vi "Set Result.vi"(8 "error in (no error)":errorcluster, 10 "XY Plot":refnum<vi>, 11 "3way Lap in":refnum<class "3way Lap.lvclass">) -> (0 "error out":errorcluster, 3 "3way Lap out":refnum<class "3way Lap.lvclass">)   [LabVIEW 2025, in "Flow Grind.lvlib" / "3way Lap.lvclass"]
uses:
  3way Lap.lvclass
  FG configuration/FlowGrind configuration.lvclass
  3way Lap.lvclass/3way Lap.ctl
  FG configuration/FlowGrind configuration.lvclass/FlowGrind configuration.ctl
  FG configuration/Read FlowGrind.vi
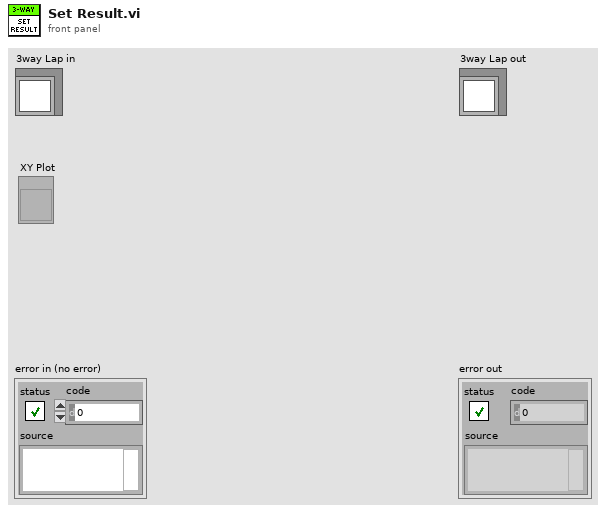
[diagram p1: front panel]
types:
  T1 = cluster{"Name":string, "Color":u32, "Style":u8, "Point Style":u8, "Name Visible":bool, "Allow Drag":bool, "Annotation Mode":u32, "Plot":i32, "Index":i32, "Position":cluster{"X":dbl, "Y":dbl}, "X Scale":u32, "Y Scale":u32, "Show Arrow":bool, "Lock Name":bool, "Plot Area":i32, "Label Offset":cluster{"X":dbl, "Y":dbl}}
  T2 = typedef "Flow Grind.lvlib/FlowGrind configuration.lvclass/FlowGrind Settings.ctl" = cluster{"Build Profile":cluster{"Ramp Start":dbl, "Ramp End":dbl, "Ramp Rate Far":dbl, "Ramp Rate Close":dbl, "Null Lower Limit":dbl, "Null Upper Limit":dbl, "Test Mode":string}[][], "Scale Factor":cluster{"X":dbl, "Y":dbl}, "Lap Condition":dbl, "Supply Pressure":dbl, "Simulated?":bool}
  T3 = typedef "LVAnnotationListTypeDef.ctl" = cluster{"Name":string, "Color":u32, "Style":u8, "Point Style":u8, "Name Visible":bool, "Allow Drag":bool, "Annotation Mode":u32, "Plot":i32, "Index":i32, "Position":cluster{"X":dbl, "Y":dbl}, "X Scale":u32, "Y Scale":u32, "Show Arrow":bool, "Lock Name":bool, "Plot Area":i32, "Label Offset":cluster{"X":dbl, "Y":dbl}}[]
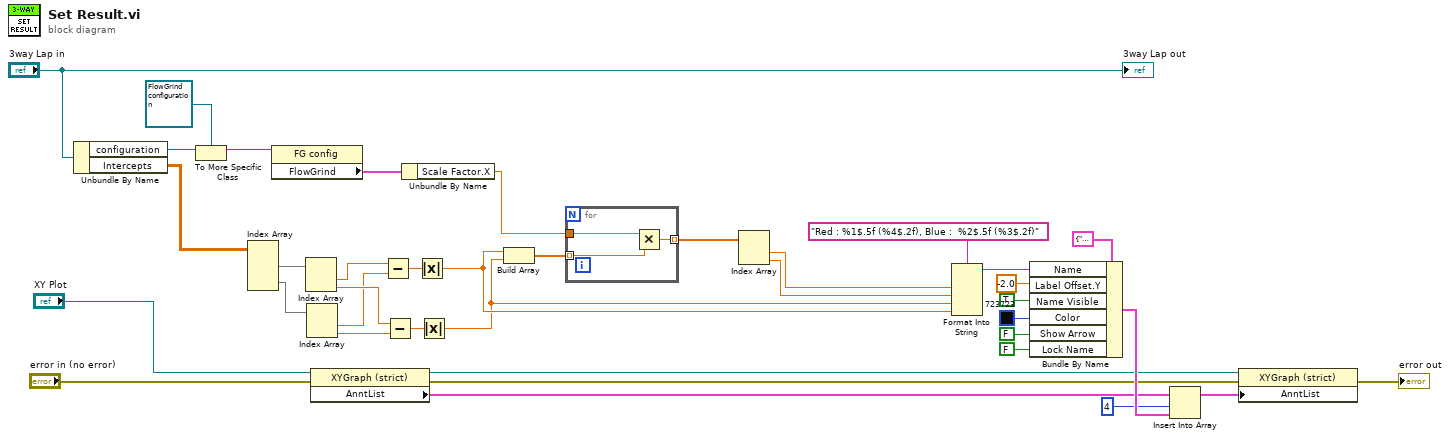
[diagram p0: block diagram]
diagram:
  n1 = Unbundle By Name("3way Lap in") -> ("configuration"=w6:refnum<class "FlowGrind configuration.lvclass">, "Intercepts"=w7:dbl[][])
  n2 = To More Specific Class(target class=refnum<class "FlowGrind configuration.lvclass"> refnum ("Flow Grind.lvlib:XY Plotter config"), reference=w6) -> (specific class reference=w4:refnum<class "FlowGrind configuration.lvclass">)  [unwired: 1 in, 1 out]
  n3 = Index Array(array=w7) -> (element #1=w13:dbl[], element #2=w14:dbl[])  [unwired: 4 in]
  n4 = property class="FG config"(reference=w4) -> ("FlowGrind"=w3:T2)  [unwired: 1 in, 2 out]
  n5 = Index Array(array=w13) -> (element #1=w15:dbl, element #2=w17:dbl)  [unwired: 2 in]
  n6 = Index Array(array=w14) -> (element #1=w16:dbl, element #2=w18:dbl)  [unwired: 2 in]
  n7 = property class="XYGraph (strict)"(reference="XY Plot", error in="error in (no error)") -> (reference out=w32:refnum<vi>, error out=w34:errorcluster, "AnntList"=w33:T3)
  n8 = Subtract(x=w15, y=w16) -> (x-y=w19:dbl)
  n9 = Subtract(x=w17, y=w18) -> (x-y=w20:dbl)
  n10 = Unbundle By Name(w3) -> ("Scale Factor.X"=w2:dbl)
  n11 = Absolute Value(x=w19) -> (abs(x)=w30:dbl)
  n12 = Absolute Value(x=w20) -> (abs(x)=w29:dbl)
  n13 = Build Array(w30, w29) -> (w11:dbl[])
  n14 = for {
    tunnel: w11 -> [w39] mode=indexing
    tunnel: w2 -> [w41]
    tunnel: [w40] -> w31 mode=indexing
    n15 = Multiply(x=w41, y=w39) -> (x*y=w40:dbl)
  }
  n16 = Index Array(array=w31) -> (element #1=w27:dbl, element #2=w28:dbl)  [unwired: 2 in]
  n17 = Format Into String(format string="Red : %1$.5f (%4$.2f), Blue :  %2$.5f (%3$.2f)", w27, w28, w29, w30) -> (resulting string=w26:string)  [unwired: 2 in, 1 out]
  n18 = Bundle By Name(cluster=T1 {"Name"="", "Color"=0, "Style"=0, "Point Style"=0, "Name Visible"=FALSE, "Allow Drag"=FALSE, "Annotation Mode"=0, "Plot"=0, "Index"=0, "Position"={"X"=0.0, "Y"=0.0}, "X Scale"=0, "Y Scale"=0, "Show Arrow"=FALSE, "Lock Name"=FALSE, "Plot Area"=0, "Label Offset"={"X"=0.0, "Y"=0.0}} ("new element/subarray"), "Name"=w26, "Label Offset.Y"=-2.0, "Name Visible"=TRUE, "Color"=u32 723723, "Show Arrow"=FALSE, "Lock Name"=FALSE) -> (w37:T1)
  n19 = Insert Into Array(array=w33, index=4, new element=w37) -> (w35:T3)
  n20 = property class="XYGraph (strict)"(reference=w32, error in=w34, "AnntList"=w35) -> (error out=→"error out":errorcluster)  [unwired: 1 out]
  "3way Lap out" <- "3way Lap in"
